vi "RDC-saltwater-generate_perm_param_to_share.vi"(11 "Stop Temp":dbl=40.0) -> (0 "used temp":dbl)   [LabVIEW 2020, in "RDC-Reflection_Data_Computation.lvlib"]
doc: "Formats the salt water model parameters per temperature, up to Stop Temp, into a text table on the panel."
uses:
  RDC-Reflection_Data_Computation.lvlib
  RDC-saltwater-param.ctl
panel:
  out "Array":T1[](array[typedef])
  out "String":string
  in  "Increment temp":dbl=5.0
  in  "Start temp":dbl=10.0
  out "unsigned 16bit integer":i32
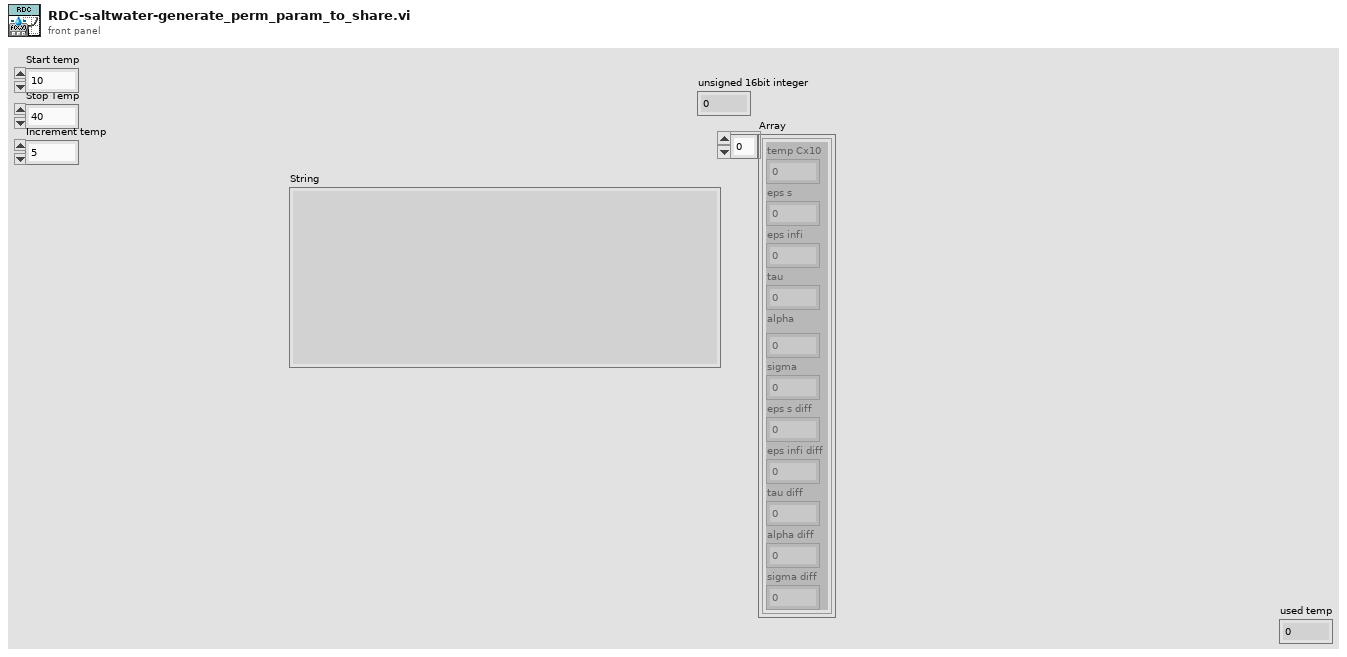
[diagram p1: front panel]
types:
  T1 = typedef "RDC-Reflection_Data_Computation.lvlib/RDC-saltwater-param.ctl" = cluster{"temp Cx10":u16, "eps s":dbl, "eps infi":dbl, "tau":dbl, "alpha":dbl, "sigma":dbl, "eps s diff":dbl, "eps infi diff":dbl, "tau diff":dbl, "alpha diff":dbl, "sigma diff":dbl}
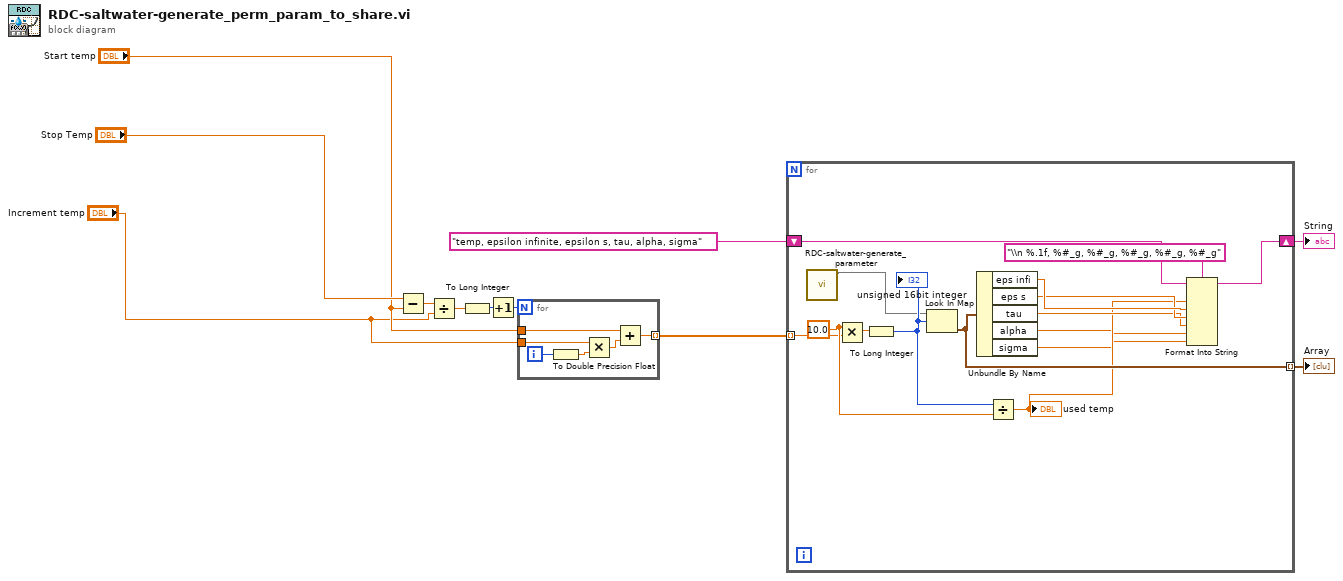
[diagram p0: block diagram]
diagram:
  n1 = Subtract(x="Stop Temp", y="Start temp") -> (x-y=w11:dbl)
  n2 = Divide(x=w11, y="Increment temp") -> (x/y=w10:dbl)
  n3 = To Long Integer(number=w10) -> (32bit integer=w9:i32)
  n4 = Increment(x=w9) -> (x+1=w8:i32)
  n5 = for {
    N: w8 -> [_]
    tunnel: "Start temp" -> [w15]
    tunnel: "Increment temp" -> [w14]
    tunnel: [w12] -> w4 mode=indexing
    i -> [w13]
    n6 = To Double Precision Float(number=w13) -> (double precision float=w17:dbl)
    n7 = Multiply(x=w14, y=w17) -> (x*y=w16:dbl)
    n8 = Add(x=w15, y=w16) -> (x+y=w12:dbl)
  }
  n9 = for {
    tunnel: w4 -> [w29] mode=indexing
    shift-right: [w28] -> w2
    shift-left: "temp, epsilon infinite, epsilon s, tau, alpha, sigma" -> [w27]
    tunnel: [w22] -> w1 mode=indexing
    w30 = 10.0 ("x")
    n10 = call "RDC-saltwater-generate_parameter.vi"() -> ("map"=w20:map{i32, T1})  [unwired: 10 in, 1 out]
    n11 = Multiply(x=w30, y=w29) -> (x*y=w32:dbl)
    n12 = To Long Integer(number=w32) -> (32bit integer=w31:i32)
    "unsigned 16bit integer" <- w31
    n13 = Look In Map(map=w20, key=w31) -> (value=w22:T1)  [unwired: 1 in, 1 out]
    n14 = Unbundle By Name(w22) -> ("eps infi"=w25:dbl, "eps s"=w24:dbl, "tau"=w23:dbl, "alpha"=w19:dbl, "sigma"=w18:dbl)
    n15 = Divide(x=w31, y=w30) -> (x/y=w21:dbl)
    "used temp" <- w21
    n16 = Format Into String(format string="\\n %.1f, %#_g, %#_g, %#_g, %#_g, %#_g", initial string=w27, w21, w25, w24, w23, w19, w18) -> (resulting string=w28:string)  [unwired: 1 in, 1 out]
  }
  "String" <- w2
  "Array" <- w1
